vi "Get_MultiVar_Values.vi"(8 "error in (no error)":errorcluster, 10 "varNames":string[](array[string]), 11 "muExpr in":refnum<class "mupExpr.lvclass">) -> (0 "error out":errorcluster, 2 "Values":dbl[](array[numeric]), 3 "muExpr out":refnum<class "mupExpr.lvclass">)   [LabVIEW 2015, in "mupExpr.lvclass"]
doc: "Lookup multiple variable values by name."
uses:
  mupExpr.lvclass
  mupExpr.lvclass/mupExpr.ctl
  <vilib>/Utility/error.llb/Error Cluster From Error Code.vi
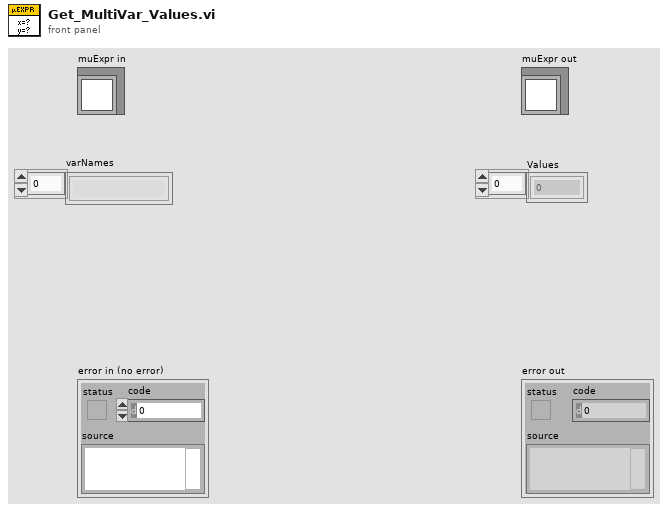
[diagram p1: front panel]
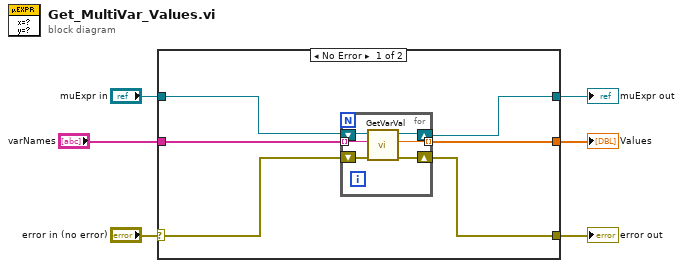
[diagram p0: block diagram]
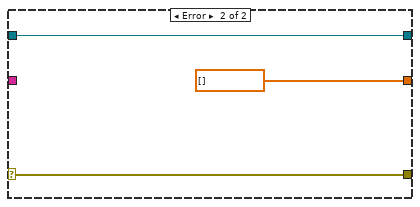
[diagram p2: hidden frame]
diagram:
  n1 = case shown="No Error" "error in (no error)" {
    selector: "error in (no error)" -> [w8 w21]
    tunnel: [w7 w21] -> w5
    tunnel: [w9 w20] -> w3
    tunnel: "muExpr in" -> [w10 w20]
    tunnel: [w12 dbl[] [] ("pd")] -> w2
    tunnel: "varNames" -> [w11 _]
    frame No Error {
      n2 = for {
        tunnel: [w14] -> w12 mode=indexing
        shift-right: [w15] -> w7
        shift-left: w8 -> [w16]
        tunnel: w11 -> [w17] mode=indexing
        shift-right: [w13] -> w9
        shift-left: w10 -> [w18]
        n3 = call "GetVarVal.vi"("error in (no error)"=w16, "varName"=w17, "muExpr in"=w18) -> ("error out"=w15:errorcluster, "varValue"=w14:dbl, "muExpr out"=w13:refnum<class "mupExpr.lvclass">)  [unwired: 6 in]
      }
    }
    frame Error {
    }
  }
  "error out" <- w5
  "muExpr out" <- w3
  "Values" <- w2
